vi "ESP32 Firmware version.vi"(8 "error in":errorcluster) -> (0 "error out":errorcluster, 1 "Command Response":string, 2 "Result":string, 3 "RESULT":bool)   [LabVIEW 2021]
uses:
  DUT/DUT_Cmd.ctl
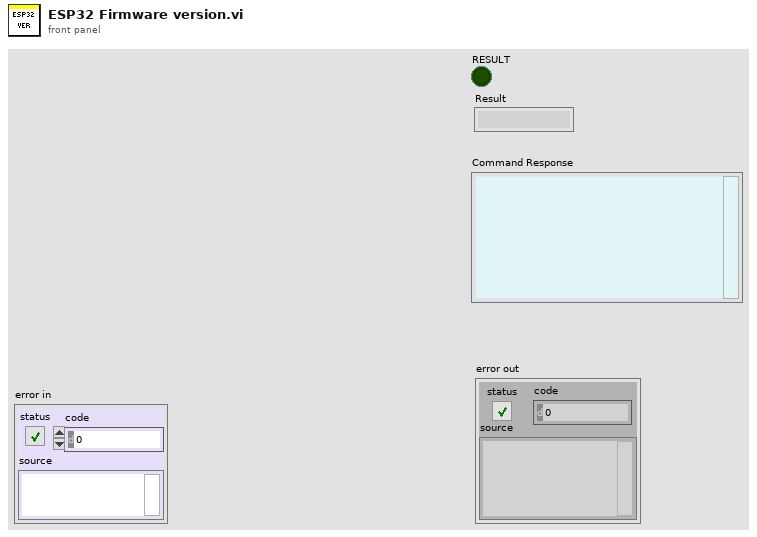
[diagram p1: front panel]
types:
  T1 = typedef "DUT_Cmd.ctl" = enum16{"Unlock serial", "Stop console logs", "Release emergency at start", "Read firmware", "WiFi credentials", "WiFi connected", "WiFi SSID", "Board revision", "ADC_NTC_TEMP", "ADC_TYPE2_RCD_CURRENT", "PCBA serial write", "PCBA serial readback", "Start energy meter", "Energy meter Vac", "Energy meter Iac", "Energy meter PF", "Energy meter energy", "Provision", "Set gateway identity", "CP checklist", "Earth detect", "D+M sense unplugged", "D+M sense plugged", "Output relay weld", "Start diagnostics", "Relay 1 on", "Relay 2 on", "Emergency pressed", "Release emergency", "Emergency released", "Unlock serial for 5 A", "Board current (5 A)", "Unlock serial for 15 A", "Board current (15 A)", "Unlock serial for 0 A", "NFC tag", "Start diagnostics again", "Relay 2 off", "Relay 1 off", "End diagnostics", "Load current (5 A) [No USB station]", "Load current (15 A) [No USB station]", "Load current (0 A) [No USB station]", "NFC tag [No USB station]", "Battery Voltage", "FW Power reset", "Notification LED", "O/P Relay weld Detection", "Earth Detection", "12V ", "5V", "3.3V", "Reboot"}
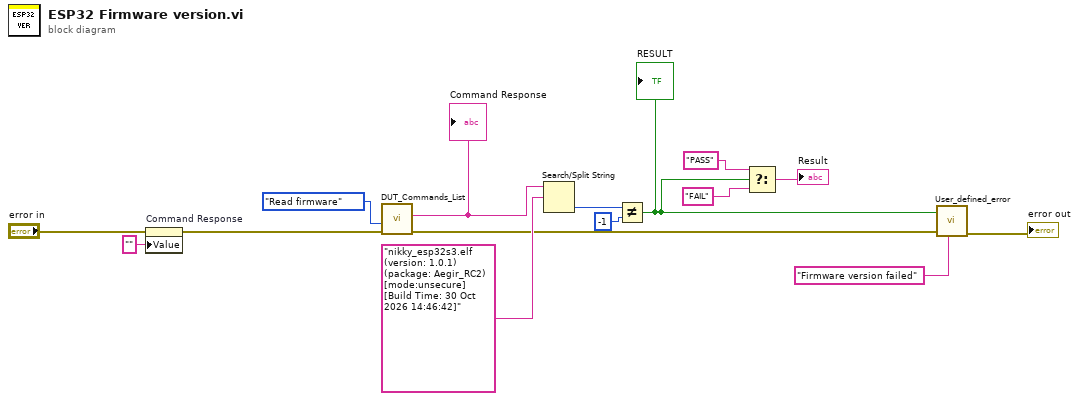
[diagram p0: block diagram]
diagram:
  n1 = property on="Command Response" class="Str"(error in="error in", "Value"="" ("Command Response")) -> (error out=w2:errorcluster)  [unwired: 1 in, 1 out]
  n2 = call "DUT_Commands_List.vi"("error in"=w2, "DUT Cmd"=DUT_Cmd."Read firmware") -> ("error out"=w5:errorcluster, "Command Response"=w4:string)  [unwired: 7 in, 1 out]
  "Command Response" <- w4
  n3 = Search/Split String(string=w4, search string/char (-)="nikky_esp32s3.elf (version: 1.0.1) (package: Aegir_RC2) [mode:unsecure] [Build Time: 30 Oct 2026 14:46:42]") -> (offset of match=w13:i32)  [unwired: 1 in, 2 out]
  n4 = Not Equal?(x=w13, y=-1) -> (x != y?=w9:bool)
  "RESULT" <- w9
  n5 = Select(t="PASS", s=w9, f="FAIL") -> (s? t:f=→"Result":string)
  n6 = call "User_defined_error.vi"("Error Msg"="Firmware version failed" ("source"), "error in"=w5, "Result"=w9) -> ("error Out"=→"error out":errorcluster)  [unwired: 8 in]
